vi "Event_Log_Loop.vi"(8 "error in (no error)":errorcluster={"status"=FALSE, "code"=0, "source"="\"\""}, 10 "file/session config":string, 11 "EventRecord queue":string) -> (0 "error out":errorcluster={"status"=FALSE, "code"=0, "source"="\"\""}, 2 "status ok":bool, 3 "Durable log status":string)   [LabVIEW 2026]
doc: "INTENT: Write all system audit events. LOGIC: Batch bounded event records to append-only storage with run and timestamp; signal backlog/disk failure."
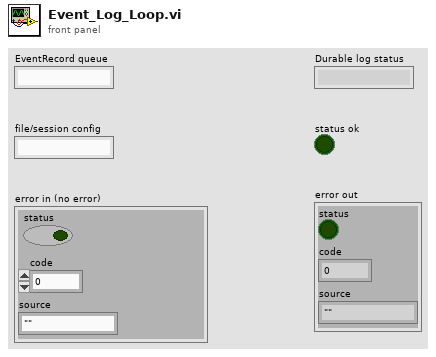
[diagram p1: front panel]
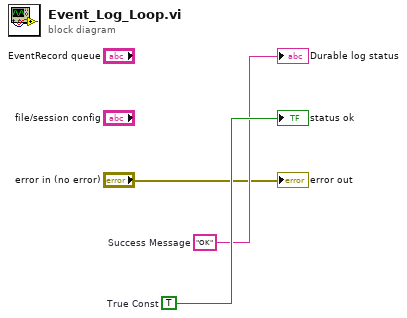
[diagram p0: block diagram]
diagram:
  w3 = TRUE  # True Const
  w2 = "OK"  # Success Message
  "Durable log status" <- w2
  "status ok" <- w3
  "error out" <- "error in (no error)"
